vi "SSL_Connect.vi"(8 "error in (no error)":errorcluster, 10 "SSL_Connection":T1, 11 "login":T2={"server IP"="", "server port"=0, "local port (0 = auto)"=0, "timeout ms (1000)"=1000}) -> (0 "error out":errorcluster, 2 "SSL_Connection":T1)   [LabVIEW 2015, in "AWS_IoT.lvlib"]
uses:
  AWS_IoT.lvlib
  Controls/SSL_login.ctl
  Controls/SSL_Connection.ctl
  <vilib>/httpClient/LabVIEWHTTPClient.lvlib
panel:
  out "Numeric":i32
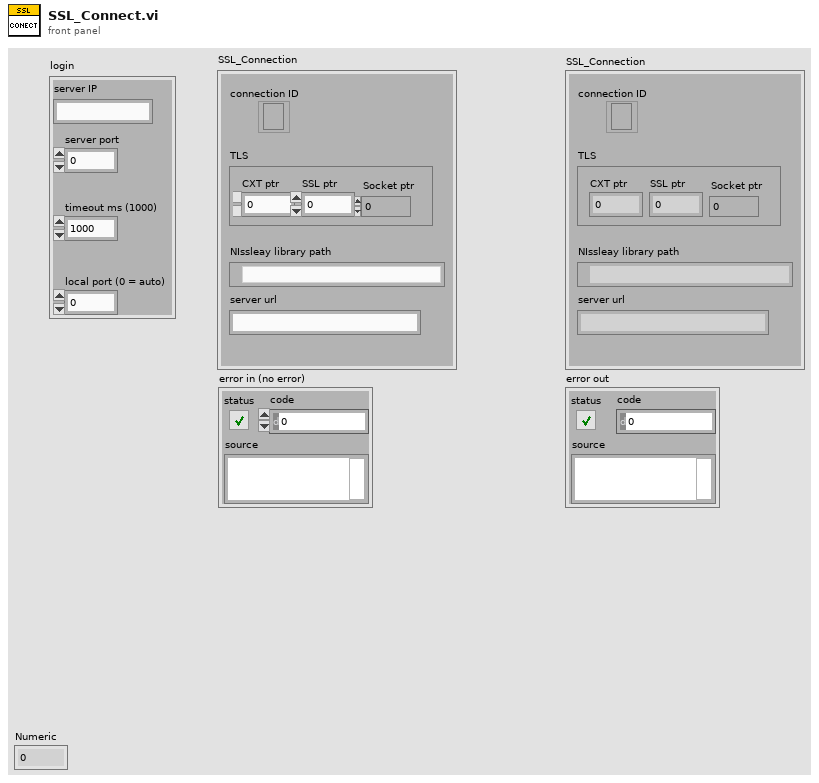
[diagram p1: front panel]
types:
  T1 = typedef "AWS_IoT.lvlib/SSL_Connection.ctl" = cluster{"connection ID":refnum<k5>, "TLS":cluster{"CXT ptr":i32, "SSL ptr":i32, "Socket ptr":i32}, "NIssleay library path":path, "server url":string}
  T2 = typedef "AWS_IoT.lvlib/SSL_login.ctl" = cluster{"server IP":string, "server port":u16, "local port (0 = auto)":u16, "timeout ms (1000)":i32}
  T3 = typedef "LabVIEWHTTPClient.lvlib/ClientHandle.ctl" = refnum<k1>
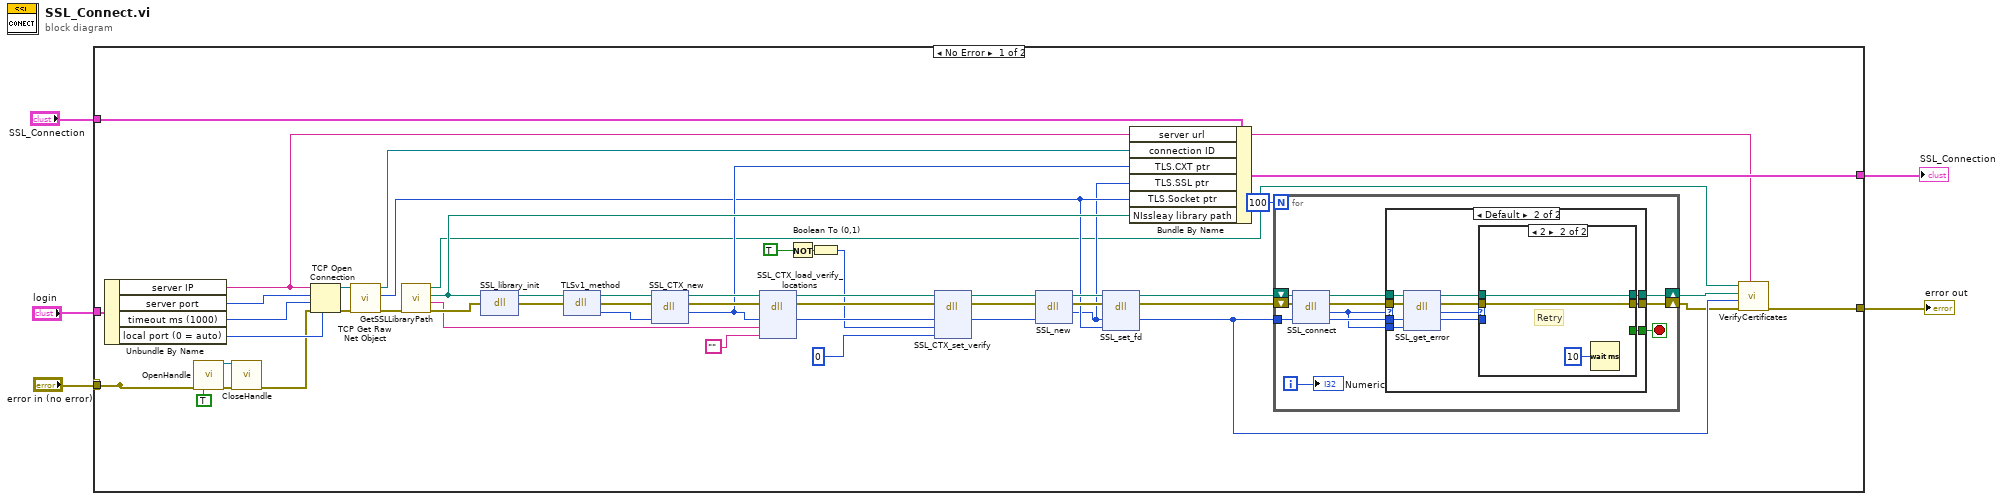
[diagram p0: block diagram]
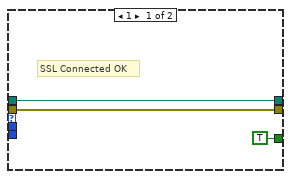
[diagram p2: hidden frame]
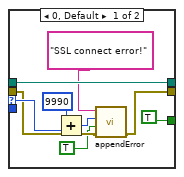
[diagram p3: hidden frame]
diagram:
  n1 = case shown="No Error" "error in (no error)" {
    selector: "error in (no error)" -> [w17 w93]
    tunnel: "login" -> [w50 _]
    tunnel: "SSL_Connection" -> [w49 w94]
    tunnel: [w20 w94] -> w3
    tunnel: [w17 _] -> _
    tunnel: [w10 w93] -> w2
    frame No Error {
      n2 = Unbundle By Name(w50) -> ("server IP"=w11:string, "server port"=w53:u16, "timeout ms (1000)"=w52:i32, "local port (0 = auto)"=w51:u16)
      n3 = call <vilib>:"OpenHandle.vi"("error in (no error)"=w17, "verify server(true)"=TRUE) -> ("client handle out"=w19:T3, "error out"=w18:errorcluster)  [unwired: 12 in]
      n4 = call <vilib>:"CloseHandle.vi"("client handle"=w19, "error in (no error)"=w18) -> ("error out"=w16:errorcluster)  [unwired: 13 in]
      n5 = TCP Open Connection(address=w11, remote port or service name=w53, timeout ms (60000)=w52, local port=w51, error in (no error)=w16) -> (connection ID=w55:refnum<k5>, error out=w54:errorcluster)
      n6 = call <vilib>:"TCP Get Raw Net Object.vi"("error in (no error)"=w54, "connection ID"=w55) -> ("error out"=w30:errorcluster, "raw net object"=w25:u64, "connection ID out"=w48:refnum<k5>)  [unwired: 7 in]
      n7 = call "GetSSLLibraryPath.vi"("error in (no error)"=w30) -> ("error out"=w28:errorcluster, "CA-bundle.crt"=w27:string, "NIssleay library path"=w29:path, "NIlibeay library pat"=w7:path)  [unwired: 7 in]
      n8 = dll-call lib="NIssleay32.*" fn="SSL_library_init"(path in=w29, error in=w28) -> (path out=w36:path, error out=w31:errorcluster)  [unwired: 2 in]
      n9 = dll-call lib="NIssleay32.*" fn="TLSv1_method"(path in=w36, error in=w31) -> (path out=w37:path, error out=w32:errorcluster, "return type"=w33:i32)  [unwired: 1 in]
      n10 = dll-call lib="NIssleay32.*" fn="SSL_CTX_new"(path in=w37, error in=w32, "ClientMethod"=w33) -> (path out=w46:path, error out=w44:errorcluster, "return type"=w26:i32)  [unwired: 2 in]
      n11 = dll-call lib="NIssleay32.*" fn="SSL_CTX_load_verify_locations"(path in=w46, error in=w44, "CTX"=w26, "CAfile"=w27, "CApath"="") -> (path out=w47:path, error out=w45:errorcluster, "CTX"=w42:i32)  [unwired: 4 in]
      n12 = Not(x=TRUE) -> (.not. x?=w23:bool)
      n13 = Boolean To (0,1)(Boolean=w23) -> (0, 1=w21:i16)
      n14 = dll-call lib="NIssleay32.*" fn="SSL_CTX_set_verify"(path in=w47, error in=w45, "CTX"=w42, "mode"=w21, "verify_callback"=0) -> (path out=w38:path, error out=w39:errorcluster, "CTX"=w40:i32)  [unwired: 4 in]
      n15 = dll-call lib="NIssleay32.*" fn="SSL_new"(path in=w38, error in=w39, "Context"=w40) -> (path out=w34:path, error out=w35:errorcluster, "return type"=w24:i32)  [unwired: 2 in]
      n16 = dll-call lib="NIssleay32.*" fn="SSL_set_fd"(path in=w34, error in=w35, "SSL"=w24, "Socket"=w25) -> (path out=w14:path, error out=w13:errorcluster, "SSL"=w9:i32)  [unwired: 3 in]
      n17 = Bundle By Name(cluster=w49, "server url"=w11, "connection ID"=w48, "TLS.CXT ptr"=w26, "TLS.SSL ptr"=w24, "TLS.Socket ptr"=w25, "NIssleay library path"=w29) -> (w20:T1)
      n18 = for {
        N: 100 -> [_]
        shift-right: [w57] -> w12
        shift-left: w14 -> [w65]
        shift-right: [w62] -> w8
        shift-left: w13 -> [w66]
        tunnel: w9 -> [w56]
        i -> [w61]
        stop <- w60 stop-if-true
        n19 = dll-call lib="NIssleay32.*" fn="SSL_connect"(path in=w65, error in=w66, "SSL"=w56) -> (path out=w64:path, error out=w63:errorcluster, "return type"=w58:i32, "SSL"=w59:i32)  [unwired: 1 in]
        n20 = case shown="Default" w58 {
          tunnel: w58 -> [_ w80]
          tunnel: w64 -> [w69 w79]
          tunnel: w63 -> [w68 w78]
          tunnel: [w68 w74] -> w62
          tunnel: [TRUE w72] -> w60
          tunnel: w59 -> [_ w71]
          tunnel: [w69 w75] -> w57
          frame 1 {
            # "SSL Connected OK"
          }
          frame Default {
            n21 = dll-call lib="NIssleay32.*" fn="SSL_get_error"(path in=w79, error in=w78, "SSL"=w71, "retCode"=w80) -> (path out=w76:path, error out=w77:errorcluster, "return type"=w73:i32, "SSL"=w70:i32)  [unwired: 2 in]
            n22 = case shown="2" w73 {
              selector: w73 -> [w87 _]
              tunnel: w77 -> [w83 w90]
              tunnel: w76 -> [w89 w91]
              tunnel: [w89 w91] -> w75
              tunnel: [w84 w90] -> w74
              tunnel: [TRUE _] -> w72
              tunnel: w70 -> [_ _]
              frame 0, Default {
                n23 = Add(x=9990, y=w87) -> (x+y=w85:i32)
                n24 = call "appendError.vi"("error in (no error)"=w83, "Boolean"=TRUE, "code"=w85, "String"="SSL connect error!" ("error message (\"\")")) -> ("error out"=w84:errorcluster)  [unwired: 7 in]
              }
              frame 2 {
                # "Retry"
                n25 = Wait (ms)(milliseconds to wait=u32 10) -> ()  [unwired: 1 out]
              }
            }
          }
        }
        "Numeric" <- w61
      }
      n26 = call "VerifyCertificates.vi"("server url"=w11, "error in (no error)"=w8, "SSL ref"=w9, "NIssleay path"=w12, "NIlibeay path"=w7) -> ("error out"=w10:errorcluster)  [unwired: 6 in]
    }
    frame Error {
    }
  }
  "SSL_Connection" <- w3
  "error out" <- w2
